vi "Kinect - Control Cluster (SubVI).vi"(7 "error in":errorcluster, 8 "Calibrate Pitch":bool, 9 "Weak detect":bool, 10 "Array of Joint Positions in":dbl[][](array[numeric])=[[-0.1347254365682602, -0.08132069557905197, 1.9283822774887085], [-0.13885043561458588, -0.016961583867669106, 2.011981248855591], [-0.14481712877750397, 0.43931880593299866, 2.1406660079956055], [-0.141028493642807, 0.6465446352958679, 2.1821846961975098], [-0.30089935660362244, 0.32630765438079834, 2.0420639514923096], [-0.26517531275749207, 0.1817575842142105, 1.7472813129425049], [-0.12027974426746368, 0.18339265882968903, 1.4648816585540771], [-0.08502443134784698, 0.17742732167243958, 1.430349588394165], [-0.003267590655013919, 0.3257020115852356, 2.05509090423584], [0.025156527757644653, 0.16852739453315735, 1.7666873931884766], [-0.0971737802028656, 0.17441977560520172, 1.473292350769043], [-0.1705384999513626, 0.18324872851371765, 1.465440034866333], [-0.21323969960212708, -0.14314982295036316, 1.8959753513336182], [-0.2711157202720642, -0.4896538555622101, 1.8643081188201904], [-0.25042033195495605, -0.8901764750480652, 1.868118405342102], [-0.23817336559295654, -0.9496505260467529, 1.7813631296157837], [-0.05292607098817825, -0.14255109429359436, 1.9082472324371338], [-0.03935781121253967, -0.4929194450378418, 1.869278073310852], [-0.03272760659456253, -0.8968366384506226, 1.8476512432098389], [-0.02717301808297634, -0.9465184211730957, 1.7542997598648071]]) -> (0 "error out":errorcluster, 2 "Control Cluster out":T1={"Roll"=0.09503769, "Pitch"=0.11711881, "Vertical Speed"=0.0, "Yaw Speed"=-0.05722916} {"Yaw Speed" scale=-1.0..1.0; "Vertical Speed" scale=-1.0..1.0; "Pitch" scale=-1.0..1.0; "Roll" scale=-1.0..1.0}, 3 "Array of Joint Positions out":dbl[][](array[numeric])=[[-0.1347254365682602, -0.08132069557905197, 1.9283822774887085], [-0.13885043561458588, -0.016961583867669106, 2.011981248855591], [-0.14481712877750397, 0.43931880593299866, 2.1406660079956055], [-0.141028493642807, 0.6465446352958679, 2.1821846961975098], [-0.30089935660362244, 0.32630765438079834, 2.0420639514923096], [-0.26517531275749207, 0.1817575842142105, 1.7472813129425049], [-0.12027974426746368, 0.18339265882968903, 1.4648816585540771], [-0.08502443134784698, 0.17742732167243958, 1.430349588394165], [-0.003267590655013919, 0.3257020115852356, 2.05509090423584], [0.025156527757644653, 0.16852739453315735, 1.7666873931884766], [-0.0971737802028656, 0.17441977560520172, 1.473292350769043], [-0.1705384999513626, 0.18324872851371765, 1.465440034866333], [-0.21323969960212708, -0.14314982295036316, 1.8959753513336182], [-0.2711157202720642, -0.4896538555622101, 1.8643081188201904], [-0.25042033195495605, -0.8901764750480652, 1.868118405342102], [-0.23817336559295654, -0.9496505260467529, 1.7813631296157837], [-0.05292607098817825, -0.14255109429359436, 1.9082472324371338], [-0.03935781121253967, -0.4929194450378418, 1.869278073310852], [-0.03272760659456253, -0.8968366384506226, 1.8476512432098389], [-0.02717301808297634, -0.9465184211730957, 1.7542997598648071]])   [LabVIEW 2014]
uses:
  Resources/Others/Control cluster.ctl
panel:
  in  "Enable Vertical movement":bool
  in  "pitch offset":dbl=0.15 format="%#_13g"
  in  "roll adjust":dbl=1.5 format="%#_13g"
  # "Experiment-based values:"
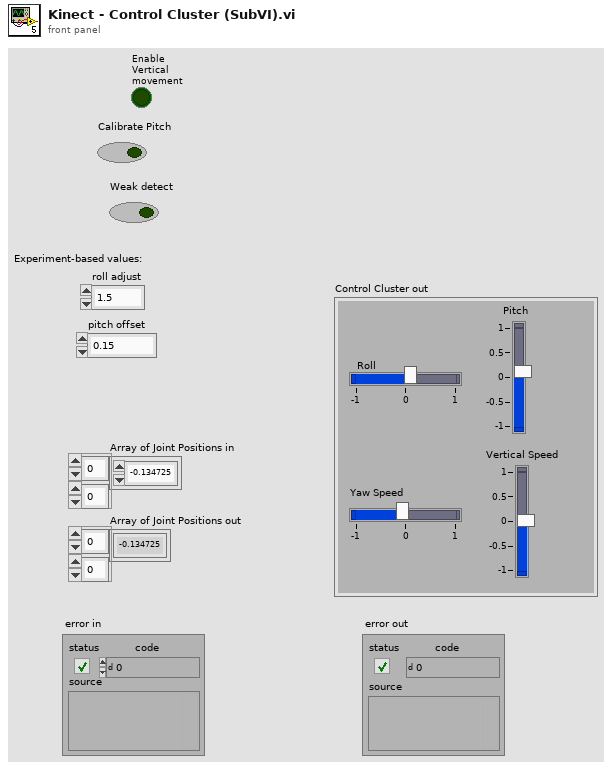
[diagram p1: front panel]
types:
  T1 = typedef "Control cluster.ctl" = cluster{"Roll":sgl, "Pitch":sgl, "Vertical Speed":sgl, "Yaw Speed":sgl}
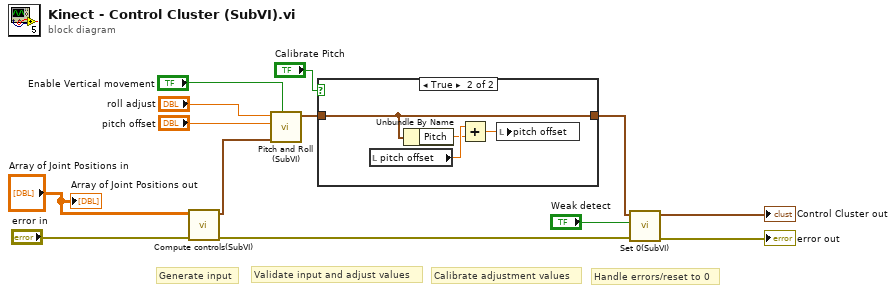
[diagram p0: block diagram]
diagram:
  # "Calibrate adjustment values"
  # "Handle errors/reset to 0"
  # "Validate input and adjust values"
  # "Generate input"
  n1 = call "Compute controls(SubVI).vi"("error in (no error)"="error in", "Array of Joint Positions in"="Array of Joint Positions in") -> ("error out"=w2:errorcluster, "Control Cluster out"=w5:T1)  [unwired: 8 in]
  n2 = call "Pitch and Roll (SubVI).vi"("Enable Vertical movement"="Enable Vertical movement", "Control Cluster in"=w5, "pitch offset"="pitch offset", "roll adjust"="roll adjust") -> ("Control Cluster out"=w8:T1)  [unwired: 5 in]
  n3 = case shown="True" "Calibrate Pitch" {
    tunnel: w8 -> [w14 w18]
    tunnel: [w14 w18] -> w7
    frame False {
    }
    frame True {
      n4 = local read "pitch offset"() -> (w17:dbl)
      n5 = Unbundle By Name(w18) -> ("Pitch"=w16:sgl)
      n6 = Add(x=w17, y=w16) -> (x+y=w15:dbl)
      n7 = local write "pitch offset"(w15) -> ()
    }
  }
  n8 = call "Set 0(SubVI).vi"("error in (no error)"=w2, "Weak detect"="Weak detect", "Control Cluster in"=w7) -> ("error out"=→"error out":errorcluster, "Control Cluster out"=→"Control Cluster out":T1)  [unwired: 7 in]
  "Array of Joint Positions out" <- "Array of Joint Positions in"
